vi "VIH HelpGen - Create Wrapper VI - VI Properties.vi"(8 "error in":errorcluster, 10 "Target VI Refnum":refnum<vi>, 11 "Source VI Refnum":refnum<vi>) -> (0 "error out":errorcluster, 1 "Terminal Wiring Rules":u16[](array[numeric]), 2 "dup Target VI Refnum":refnum<vi>, 3 "dup Source VI Refnum":refnum<vi>)   [LabVIEW 2014]
doc: "::: VI Helpeks :::\nCopyright (c) 2000-2026 Konstantin Shifershteyn. All rights reserved."
panel:
  out "Wire Rule":T1(ring)
  # "VI Helpeks\nCopyright (c) 2012-2026 Konstantin Shifershteyn"
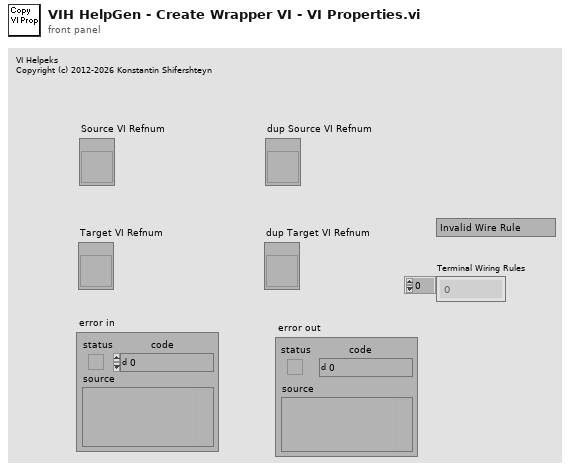
[diagram p1: front panel]
types:
  T1 = enum16{"Invalid Wire Rule", "Required", "Recommended", "Optional", "Dynamic Dispatch"}
  T2 = typedef "imagedata.ctl" = cluster{"image type":i32, "image depth":i32, "image":u8[], "mask":u8[], "colors":u32[], "Rectangle":cluster{"left":i16, "top":i16, "right":i16, "bottom":i16}}
  T3 = enum16{"Invalid Wire Rule", "Required", "Recommended", "Optional", "Dynamic Dispatch"}[]
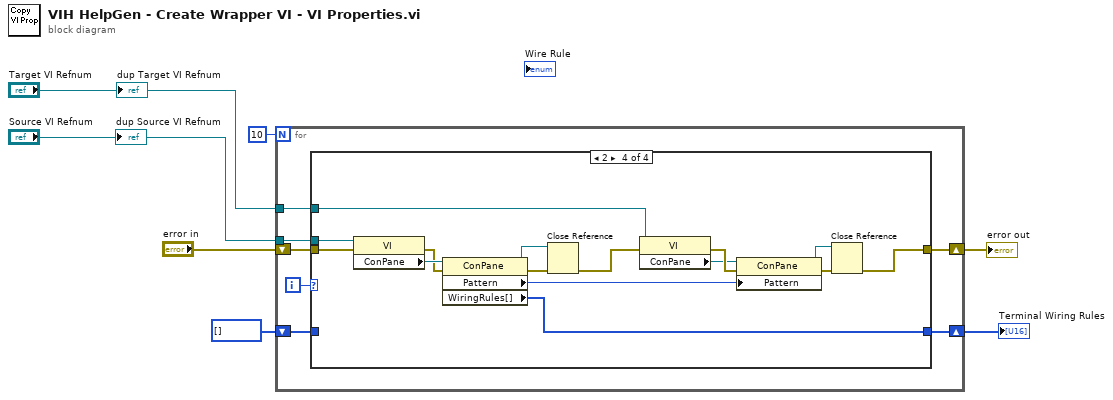
[diagram p0: block diagram]
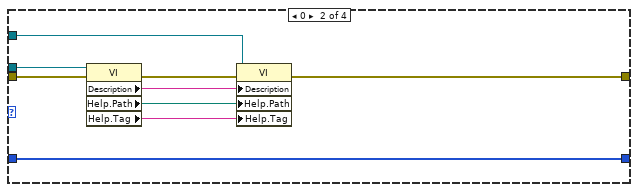
[diagram p3: hidden frame]
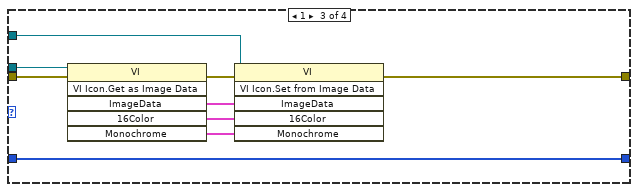
[diagram p4: hidden frame]
diagram:
  n1 = for {
    N: 10 -> [_]
    shift-right: [w12] -> w4
    shift-left: "error in" -> [w13]
    tunnel: "Source VI Refnum" -> [w11]
    tunnel: "Target VI Refnum" -> [w10]
    shift-right: [w9] -> w1
    shift-left: u16[] [] ("WiringRules[]") -> [w8]
    i -> [w14]
    n2 = case shown="2" w14 {
      tunnel: w13 -> [w16 w22 w30 w46]
      tunnel: [w16 w20 w27 w36] -> w12
      tunnel: w11 -> [_ w19 w29 w47]
      tunnel: w10 -> [_ w18 w28 w42]
      tunnel: [w15 w17 w26 w35] -> w9
      tunnel: w8 -> [w15 w17 w26 _]
      frame Default {
      }
      frame 0 {
        n3 = property class="VI"(reference=w19, error in=w22) -> (error out=w21:errorcluster, "Description"=w25:string, "Help.Path"=w24:path, "Help.Tag"=w23:string)  [unwired: 1 out]
        n4 = property class="VI"(reference=w18, error in=w21, "Description"=w25, "Help.Path"=w24, "Help.Tag"=w23) -> (error out=w20:errorcluster)  [unwired: 1 out]
      }
      frame 1 {
        n5 = invoke class="VI" method="VI Icon.Get as Image Data"(reference=w29, error in=w30) -> (error out=w34:errorcluster, "ImageData"=w31:T2, "16Color"=w32:T2, "Monochrome"=w33:T2)  [unwired: 4 in, 2 out]
        n6 = invoke class="VI" method="VI Icon.Set from Image Data"(reference=w28, error in=w34, "ImageData"=w31, "16Color"=w32, "Monochrome"=w33) -> (error out=w27:errorcluster)  [unwired: 1 in, 5 out]
      }
      frame 2 {
        n7 = property class="VI"(reference=w47, error in=w46) -> (error out=w43:errorcluster, "ConPane"=w48:refnum<vi>)  [unwired: 1 out]
        n8 = property class="ConPane"(reference=w48, error in=w43) -> (reference out=w49:refnum<vi>, error out=w40:errorcluster, "Pattern"=w41:u32, "WiringRules[]"=w35:T3)
        n9 = Close Reference(reference=w49, error in (no error)=w40) -> (error out=w39:errorcluster)
        n10 = property class="VI"(reference=w42, error in=w39) -> (error out=w45:errorcluster, "ConPane"=w44:refnum<vi>)  [unwired: 1 out]
        n11 = property class="ConPane"(reference=w44, error in=w45, "Pattern"=w41) -> (reference out=w37:refnum<vi>, error out=w38:errorcluster)
        n12 = Close Reference(reference=w37, error in (no error)=w38) -> (error out=w36:errorcluster)
      }
    }
  }
  "error out" <- w4
  "Terminal Wiring Rules" <- w1
  "dup Source VI Refnum" <- "Source VI Refnum"
  "dup Target VI Refnum" <- "Target VI Refnum"
